vi "Untitled 5.vi"() -> ()   [LabVIEW 2018]
panel:
  in  "Boolean 5":bool
  in  "Boolean 4":bool
  out "Boolean 3":bool
  in  "Boolean 2":bool
  in  "Boolean":bool
  out "Numeric 5":dbl
  in  "Numeric 3":dbl
  out "Numeric 2":dbl
  in  "Numeric":dbl
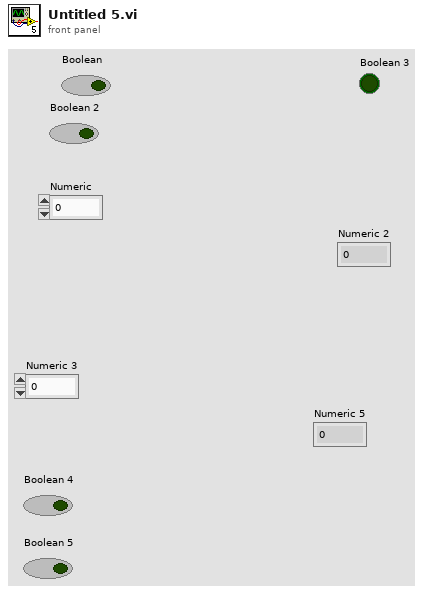
[diagram p1: front panel]
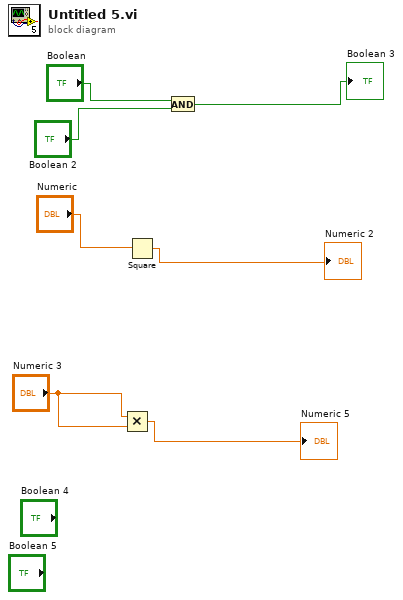
[diagram p0: block diagram]
diagram:
  n1 = Multiply(x="Numeric 3", y="Numeric 3") -> (x*y=→"Numeric 5":dbl)
  n2 = Square(x="Numeric") -> (x^2=→"Numeric 2":dbl)
  n3 = And(x="Boolean", y="Boolean 2") -> (x .and. y?=→"Boolean 3":bool)
